vi "nevstop-programming-palette - Pre-Build Custom Action.vi"(10 "Variant":variant) -> (0 "error out":errorcluster)   [LabVIEW 2017]
panel:
  out "Array":T1(array[cluster])
  out "dup Folder Path":path
  out "n":i32
  out "i":i32
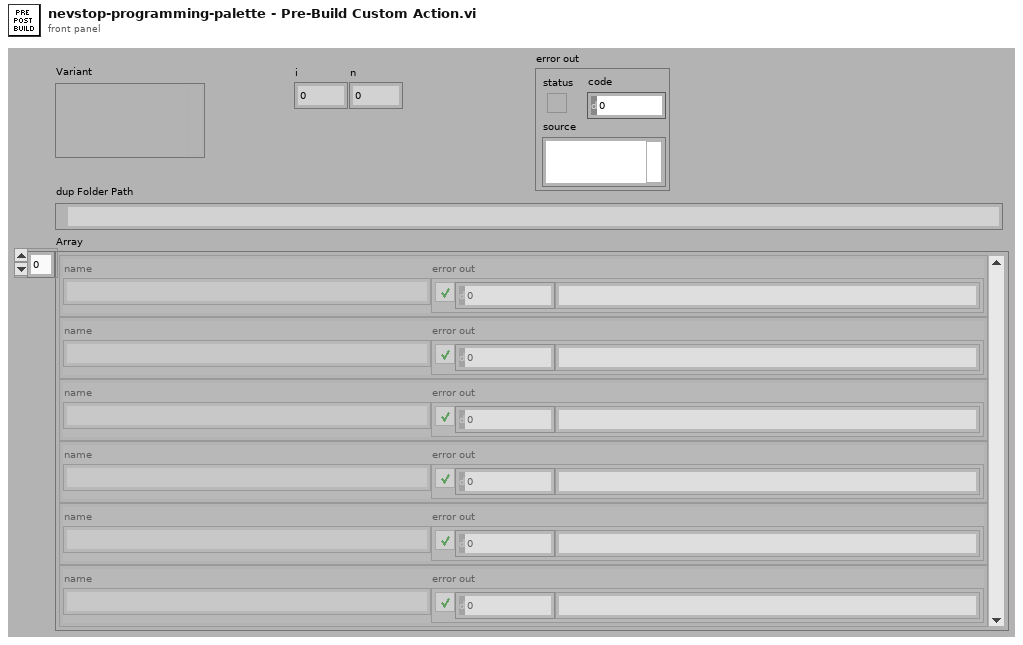
[diagram p1: front panel]
types:
  T1 = cluster{"name":string, "error out":errorcluster}[]
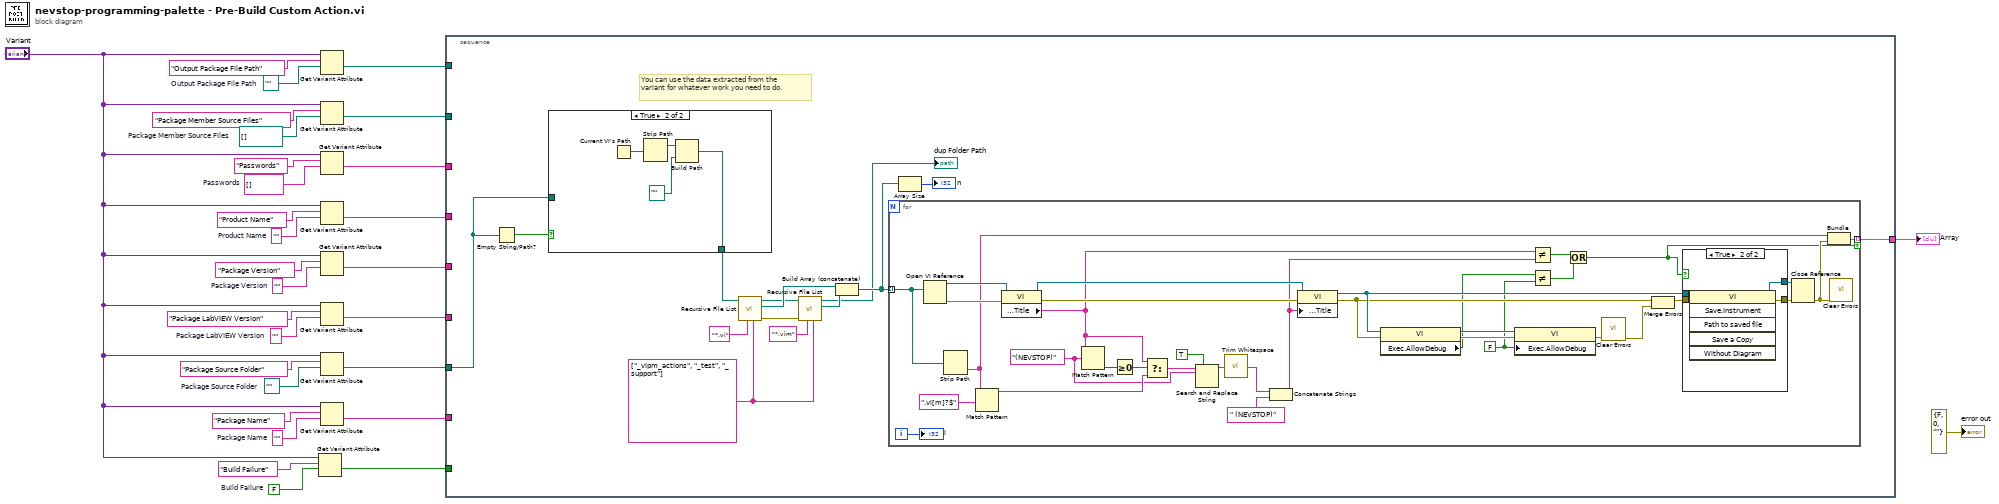
[diagram p0: block diagram]
diagram:
  w4 = FALSE  # Build Failure
  w14 = path ""  # Package Source Folder
  w15 = ""  # Package Name
  w18 = ""  # Package LabVIEW Version
  w20 = ""  # Package Version
  w22 = ""  # Product Name
  w25 = string[] []  # Passwords
  w27 = path[] []  # Package Member Source Files
  w29 = path ""  # Output Package File Path
  n1 = Get Variant Attribute(Variant="Variant", name="Build Failure", default value (empty Variant)=w4) -> (value=w2:bool)  [unwired: 1 in, 3 out]
  n2 = Get Variant Attribute(Variant="Variant", name="Output Package File Path", default value (empty Variant)=w29) -> (value=w13:path)  [unwired: 1 in, 3 out]
  n3 = Get Variant Attribute(Variant="Variant", name="Package Member Source Files", default value (empty Variant)=w27) -> (value=w12:path[])  [unwired: 1 in, 3 out]
  n4 = Get Variant Attribute(Variant="Variant", name="Passwords", default value (empty Variant)=w25) -> (value=w11:string[])  [unwired: 1 in, 3 out]
  n5 = Get Variant Attribute(Variant="Variant", name="Product Name", default value (empty Variant)=w22) -> (value=w10:string)  [unwired: 1 in, 3 out]
  n6 = Get Variant Attribute(Variant="Variant", name="Package Version", default value (empty Variant)=w20) -> (value=w9:string)  [unwired: 1 in, 3 out]
  n7 = Get Variant Attribute(Variant="Variant", name="Package LabVIEW Version", default value (empty Variant)=w18) -> (value=w8:string)  [unwired: 1 in, 3 out]
  n8 = Get Variant Attribute(Variant="Variant", name="Package Source Folder", default value (empty Variant)=w14) -> (value=w7:path)  [unwired: 1 in, 3 out]
  n9 = Get Variant Attribute(Variant="Variant", name="Package Name", default value (empty Variant)=w15) -> (value=w6:string)  [unwired: 1 in, 3 out]
  n10 = stacked-sequence {
    tunnel: w13 -> [_]
    tunnel: w12 -> [_]
    tunnel: w11 -> [_]
    tunnel: w10 -> [_]
    tunnel: w9 -> [_]
    tunnel: w8 -> [_]
    tunnel: w7 -> [w33]
    tunnel: w6 -> [_]
    tunnel: w2 -> [_]
    tunnel: [w32] -> w1
    frame #0 {
      w38 = string[] ["_vipm_actions", "_test", "_support"] ("Folders to Exclude")
      # "You can use the data extracted from the variant for whatever work you need to do."
      n11 = Empty String/Path?(string/path=w33) -> (empty?=w34:bool)
      n12 = case shown="True" w34 {
        tunnel: [w45 w46] -> w31
        tunnel: w33 -> [w45 _]
        frame False {
        }
        frame True {
          n13 = Current VI's Path() -> (path=w49:path)
          n14 = Strip Path(path=w49) -> (stripped path=w48:path)  [unwired: 1 out]
          n15 = Build Path(base path=w48, name or relative path=path ".." ("Relative path (.)")) -> (appended path=w46:path)
        }
      }
      n16 = call <vilib>:"Recursive File List.vi"("Folders to Exclude"=w38, "pattern"="*.vi", "Folder Path"=w31) -> ("error out"=w42:errorcluster, "All Files in Dir"=w41:path[], "dup Folder Path"=w39:path)  [unwired: 4 in, 2 out]
      n17 = call <vilib>:"Recursive File List.vi"("Folders to Exclude"=w38, "pattern"="*.vim", "error in (no error)"=w42, "Folder Path"=w39) -> ("All Files in Dir"=w40:path[], "dup Folder Path"=→"dup Folder Path":path)  [unwired: 3 in, 3 out]
      n18 = Build Array (concatenate)(w41, w40) -> (w37:path[])
      n19 = for {
        tunnel: w37 -> [w82] mode=indexing
        tunnel: [w67] -> w32 mode=indexing if=w50
        i -> [w80]
        w53 = FALSE ("Execution:Allow Debugging")
        w70 = "(NEVSTOP)" ("string")
        n20 = Open VI Reference(vi path=w82) -> (vi reference=w77:refnum<vi>, error out=w79:errorcluster)  [unwired: 5 in]
        n21 = Strip Path(path=w82) -> (name=w65:string)  [unwired: 1 out]
        n22 = Match Pattern(string=w65, regular expression=".vi[m]?$") -> (before substring=w72:string)  [unwired: 1 in, 3 out]
        n23 = property class="VI"(reference=w77, error in=w79) -> (reference out=w76:refnum<vi>, error out=w78:errorcluster, "Front Panel.Title"=w56:string)
        n24 = Match Pattern(string=w56, regular expression=w70) -> (offset past match=w74:i32)  [unwired: 1 in, 3 out]
        n25 = Greater Or Equal To 0?(x=w74) -> (x >= 0?=w73:bool)
        n26 = Select(t=w56, s=w73, f=w72) -> (s? t:f=w71:string)
        n27 = Search and Replace String(replace all?=TRUE ("replace all? (F)"), input string=w71, search string=w70) -> (result string=w68:string)  [unwired: 5 in, 3 out]
        n28 = call <vilib>:"Trim Whitespace.vi"("string"=w68) -> ("trimmed string"=w64:string)  [unwired: 1 in]
        n29 = Concatenate Strings(w64, " (NEVSTOP)" ("string")) -> (w55:string)
        n30 = property class="VI"(reference=w76, error in=w78, "Front Panel.Title"=w55) -> (reference out=w60:refnum<vi>, error out=w57:errorcluster)
        n31 = property class="VI"(reference=w60, error in=w57) -> (reference out=w59:refnum<vi>, error out=w58:errorcluster, "Exec.AllowDebug"=w54:bool)
        n32 = property class="VI"(reference=w59, error in=w58, "Exec.AllowDebug"=w53) -> (error out=w63:errorcluster)  [unwired: 1 out]
        n33 = Not Equal?(x=w56, y=w55) -> (x != y?=w52:bool)
        n34 = Not Equal?(x=w54, y=w53) -> (x != y?=w51:bool)
        n35 = Or(x=w52, y=w51) -> (x .or. y?=w50:bool)
        n36 = call <vilib>:"Clear Errors.vi"("error in (no error)"=w63) -> ("error out"=w61:errorcluster)  [unwired: 5 in, 1 out]
        n37 = Merge Errors(w57, w61) -> (w62:errorcluster)
        n38 = case shown="True" w50 {
          tunnel: [w85 w90] -> w84
          tunnel: [w86 w89] -> w83
          tunnel: w62 -> [w85 w88]
          tunnel: w60 -> [w86 w87]
          frame False {
          }
          frame True {
            n39 = invoke class="VI" method="Save.Instrument"(reference=w87, error in=w88) -> (reference out=w89:refnum<vi>, error out=w90:errorcluster)  [unwired: 4 in, 4 out]
          }
        }
        n40 = Close Reference(reference=w83, error in (no error)=w84) -> (error out=w66:errorcluster)
        n41 = Bundle("name"=w65, "error out"=w66) -> (w67:cluster{"name":string, "error out":errorcluster})  [unwired: 1 in]
        n42 = call <vilib>:"Clear Errors.vi"("error in (no error)"=w66) -> ()  [unwired: 5 in, 2 out]
        "i" <- w80
      }
      n43 = Array Size(array=w37) -> (size(s)=→"n":i32)
    }
  }
  "Array" <- w1
  "error out" <- errorcluster {"status"=FALSE, "code"=0, "source"=""} ("error out")
